vi "read channels of classification.vi"(6 "channel classification":T2, 8 "error in":errorcluster, 11 "Shared Memory runtime in":refnum<class "Shared Memory runtime.lvclass">) -> (0 "error out":errorcluster, 2 "channels":T1[](array[typedef]), 3 "Shared Memory runtime out":refnum<class "Shared Memory runtime.lvclass">)   [LabVIEW 2014, in "Shared Memory runtime.lvclass"]
uses:
  Shared Memory runtime.lvclass
  <vilib>/NI/Tag Bus Module Framework/channel/channel classification.ctl
  channel runtime.ctl
  <vilib>/NI/Tag Bus/tag/Data Type.ctl
  <vilib>/NI/NI Linux RT IPC/Shared Memory/Controls/reference.ctl
  <vilib>/NI/NI Linux RT IPC/Shared Memory/Classes/Shared Memory/Shared Memory.lvclass
  Shared Memory runtime.lvclass/Shared Memory runtime.ctl
  <vilib>/NI/Tag Bus Module Framework/channel/TBM channel.lvclass
  <vilib>/NI/Tag Bus/tag/tag descriptor.lvclass
  <vilib>/NI/NI Linux RT IPC/Shared Memory/Linux RT IPC.Shared Memory.lvlib
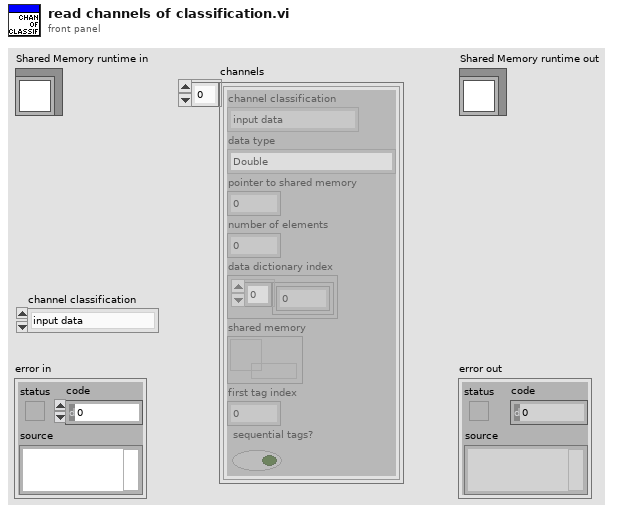
[diagram p1: front panel]
types:
  T1 = typedef "Shared Memory runtime.lvclass/channel runtime.ctl" = cluster{"channel classification":T2, "data type":T3, "pointer to shared memory":u64, "number of elements":u64, "data dictionary index":cluster{i32[]}, "shared memory":T4, "first tag index":i32, "sequential tags?":bool}
  T2 = typedef "TBM channel.lvclass/channel classification.ctl" = enum16{"input data", "output data", "processing parameter", "processing result"}
  T3 = typedef "tag bus.lvlib/tag descriptor.lvclass/Data Type.ctl" = enum16{"Double", "Single", "I64", "I32", "I16", "I8", "U64", "U32", "U16", "U8", "Boolean", "String", "Array of Double", "Array of Single", "Array of I64", "Array of I32", "Array of I16", "Array of I8", "Array of U64", "Array of U32", "Array of U16", "Array of U8", "Array of Boolean", "Array of String"}
  T4 = typedef "Linux RT IPC.Shared Memory.lvlib/reference.ctl" = refnum<data-value>
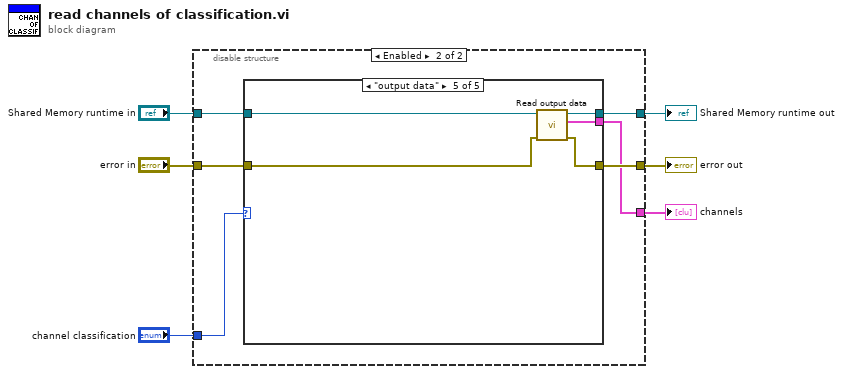
[diagram p0: block diagram]
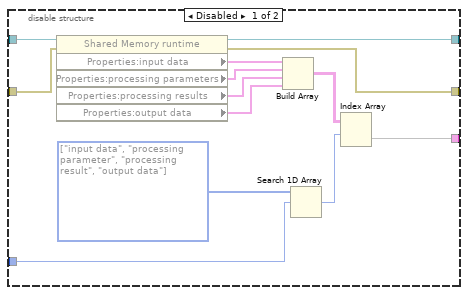
[diagram p2: hidden frame]
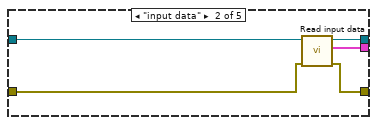
[diagram p4: hidden frame]
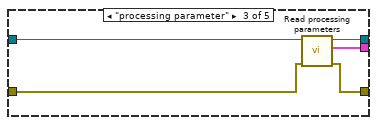
[diagram p5: hidden frame]
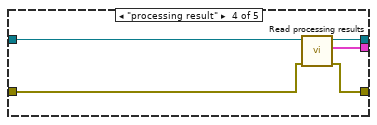
[diagram p6: hidden frame]
diagram:
  n1 = disable-structure shown="Enabled" {
    disable-tunnel: "channel classification" -> [w12 w24]
    disable-tunnel: "Shared Memory runtime in" -> [w11 w25]
    disable-tunnel: [w10 w23] -> w4
    disable-tunnel: [w9 w21] -> w3
    disable-tunnel: "error in" -> [w8 w22]
    disable-tunnel: [w7 w20] -> w1
    frame Disabled {
      w16 = T2[] [enum."input data", enum."processing parameter", enum."processing result", enum."output data"] items=["input data", "output data", "processing parameter", "processing result"] ("supported classifications")
      n2 = property class="Shared Memory runtime"(reference=w11, error in=w8) -> (reference out=w10:refnum<class "Shared Memory runtime.lvclass">, error out=w9:errorcluster, "Properties:input data"=w19:T1[], "Properties:processing parameters"=w15:T1[], "Properties:processing results"=w14:T1[], "Properties:output data"=w13:T1[])
      n3 = Build Array(w19, w15, w14, w13) -> (w17:T1[][])
      n4 = Search 1D Array(1D array=w16, element=w12) -> (index of element=w18:i32)  [unwired: 1 in]
      n5 = Index Array(array=w17, index (row)=w18) -> (element=w7:T1[])  [unwired: 1 in]
    }
    frame Enabled {
      n6 = case shown="\"output data\"" w24 {
        tunnel: w25 -> [w27 w32 w37 w42 w47]
        tunnel: [w27 w31 w36 w41 w46] -> w23
        tunnel: [_ w30 w35 w40 w43] -> w20
        tunnel: w22 -> [w26 w28 w33 w38 w44]
        tunnel: [w26 w29 w34 w39 w45] -> w21
        frame Default {
        }
        frame "input data" {
          n7 = call "Read input data.vi"("error in"=w28, "Shared Memory runtime in"=w32) -> ("error out"=w29:errorcluster, "input data"=w30:T1[], "Shared Memory runtime out"=w31:refnum<class "Shared Memory runtime.lvclass">)  [unwired: 7 in]
        }
        frame "processing parameter" {
          n8 = call "Read processing parameters.vi"("error in"=w33, "Shared Memory runtime in"=w37) -> ("error out"=w34:errorcluster, "processing parameters"=w35:T1[], "Shared Memory runtime out"=w36:refnum<class "Shared Memory runtime.lvclass">)  [unwired: 7 in]
        }
        frame "processing result" {
          n9 = call "Read processing results.vi"("error in"=w38, "Shared Memory runtime in"=w42) -> ("error out"=w39:errorcluster, "processing results"=w40:T1[], "Shared Memory runtime out"=w41:refnum<class "Shared Memory runtime.lvclass">)  [unwired: 7 in]
        }
        frame "output data" {
          n10 = call "Read output data.vi"("error in"=w44, "Shared Memory runtime in"=w47) -> ("error out"=w45:errorcluster, "output data"=w43:T1[], "Shared Memory runtime out"=w46:refnum<class "Shared Memory runtime.lvclass">)  [unwired: 7 in]
        }
      }
    }
  }
  "error out" <- w3
  "Shared Memory runtime out" <- w4
  "channels" <- w1
